vi "VHistFile - File paths from Time Array.vi"(5 "log directory":path=path "DataLog", 6 "time stamps":dbl[](array[numeric]) format="%<%H:%M:%S%2u\n%d/%m/%Y>T", 7 "file extension (.bin)":string=".bin", 8 "path pattern":T1(ring), 9 "file tag":string) -> (2 "subset info":cluster{"index":i32, "length":i32}[](array[cluster]), 3 "file paths":path[](array[path]))   [LabVIEW 2021]
doc: "::: CalcExpress Toolkit :::\nCopyright (c) 2000-2026 Konstantin Shifershteyn. All rights reserved."
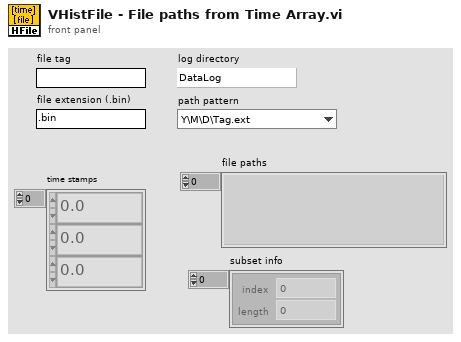
[diagram p1: front panel]
types:
  T1 = enum32{"Y\\M\\D\\Tag.ext", "Y\\M\\D\\Tag [Y-M-D].ext", "Y-M-D\\Tag.ext", "Y-M-D\\Tag [Y-M-D].ext", "Tag [Y-M-D].ext"}
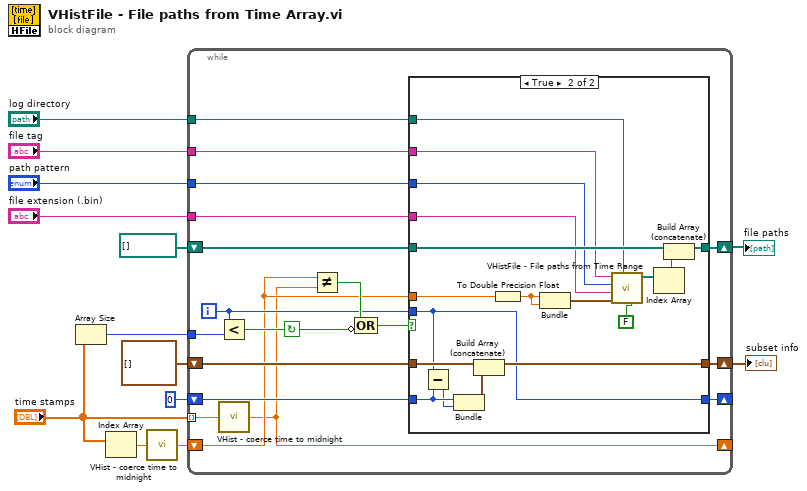
[diagram p0: block diagram]
diagram:
  n1 = Array Size(array="time stamps") -> (size(s)=w13:i32)
  n2 = Index Array(array="time stamps") -> (element=w6:dbl)  [unwired: 1 in]
  n3 = call "VHist - coerce time to midnight.vi"("time"=w6) -> ("midnight"=w5:dbl)  [unwired: 4 in]
  n4 = while {
    shift-left: path[] [] -> [w21]
    shift-right: [w22] -> w7
    tunnel: w13 -> [w30]
    shift-left: cluster{i32, i32}[] [] -> [w24]
    shift-right: [w25] -> w11
    shift-left: 0 -> [w31]
    shift-right: [w23] -> _
    shift-left: w5 -> [w20]
    shift-right: [w19] -> _
    tunnel: "time stamps" -> [w18] mode=indexing
    tunnel: "path pattern" -> [w17]
    tunnel: "file tag" -> [w16]
    tunnel: "log directory" -> [w15]
    tunnel: "file extension (.bin)" -> [w14]
    i -> [w26]
    stop <- w29 continue-if-true
    n5 = Less?(x=w26, y=w30) -> (x < y?=w29:bool)
    n6 = call "VHist - coerce time to midnight.vi"("time"=w18) -> ("midnight"=w19:dbl)  [unwired: 4 in]
    n7 = Not Equal?(x=w20, y=w19) -> (x != y?=w28:bool)
    n8 = Compound Arithmetic op=OR(w28, invert w29) -> (w27:bool)
    n9 = case shown="True" w27 {
      tunnel: w31 -> [w33 w52]
      tunnel: w26 -> [_ w47]
      tunnel: [w34 w49] -> w25
      tunnel: w24 -> [w34 w48]
      tunnel: [w33 w47] -> w23
      tunnel: [w32 w46] -> w22
      tunnel: w21 -> [w32 w43]
      tunnel: w20 -> [_ w41]
      tunnel: w17 -> [_ w38]
      tunnel: w16 -> [_ w37]
      tunnel: w15 -> [_ w36]
      tunnel: w14 -> [_ w35]
      frame False {
      }
      frame True {
        n10 = Subtract(x=w47, y=w52) -> (x-y=w51:i32)
        n11 = Bundle(w52, w51) -> (w50:cluster{i32, i32})  [unwired: 1 in]
        n12 = Build Array (concatenate)(w48, w50) -> (w49:cluster{i32, i32}[])
        n13 = To Double Precision Float(number=w41) -> (double precision float=w42:dbl)
        n14 = Bundle(w42, w42) -> (w40:cluster{dbl, dbl})  [unwired: 1 in]
        n15 = call "VHistFile - File paths from Time Range.vi"("extended range (F)"=FALSE, "log directory"=w36, "time range"=w40, "file extension (.bin)"=w35, "path pattern"=w38, "file tag"=w37) -> ("file paths"=w45:path[])  [unwired: 3 in]
        n16 = Index Array(array=w45) -> (element=w44:path)  [unwired: 1 in]
        n17 = Build Array (concatenate)(w43, w44) -> (w46:path[])
      }
    }
  }
  "file paths" <- w7
  "subset info" <- w11
